vi "FuncVI2-_Call.vi"(4 "Caller CSE RefNum":T1, 5 "InstanceRef":T3, 9 "arg list":T2[](array[typedef]) {"num" format="%.2f"}) -> (0 "error out":bool, 3 "result":T2 {"num" format="%.2f"})   [LabVIEW 2021]
doc: "::: CalcExpress Toolkit :::\nCopyright (c) 2000-2026 Konstantin Shifershteyn. All rights reserved."
uses:
  cetypes.llb/CalcExpress Function Argument Info.ctl
  cetypes.llb/CalcExpress Instance RefNum.ctl
  cse.llb/CSE Instance RefNum.ctl
panel:
  in  "max arg num":i32=1000
  in  "min arg num":i32=1
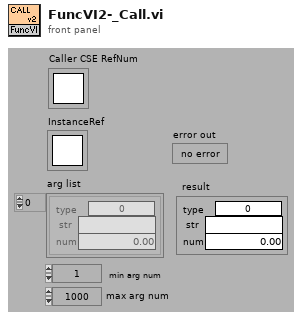
[diagram p1: front panel]
types:
  T1 = typedef "CSE Instance RefNum.ctl" = refnum<k1>
  T2 = typedef "CalcExpress Function Argument Info.ctl" = cluster{"type":u32, "str":string, "num":dbl}
  T3 = typedef "CalcExpress Instance RefNum.ctl" = refnum<k1>
  T4 = enum32{"String", "DBL Number", "identifier", "1D Array of DBL", "2D Array of DBL", "CDB Number", "1D Array of CDB", "2D Array of CDB", "1D Array of String", "2D Array of String", "Unknown data type"}
  T5 = typedef "VarMan Variable Context Handle.ctl" = i32
  T6 = typedef "CSE Callback VI RefNum.ctl" = refnum<vi>
  T7 = cluster{"type: use this constant to specify a predefined type code":enum32{"String", "DBL Number", "identifier", "1D Array of DBL", "2D Array of DBL", "CDB Number", "1D Array of CDB", "2D Array of CDB", "1D Array of String", "2D Array of String", "Unknown data type"}, string, "return value":dbl}
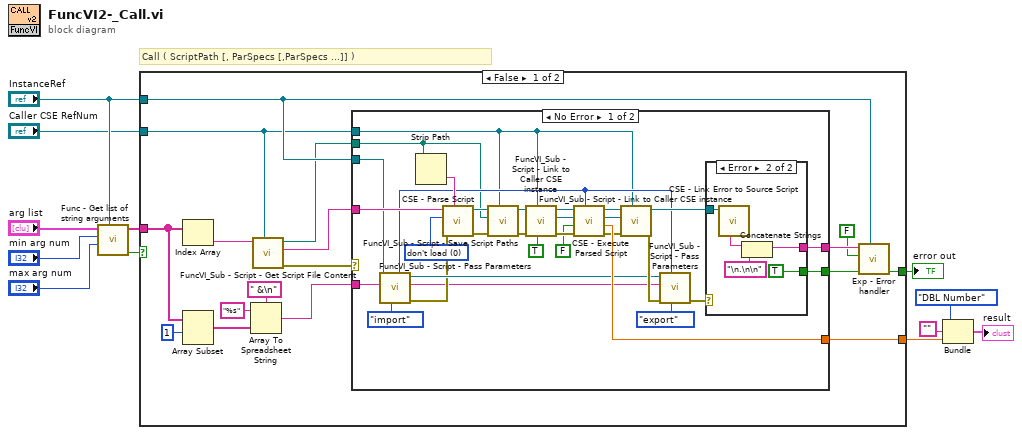
[diagram p0: block diagram]
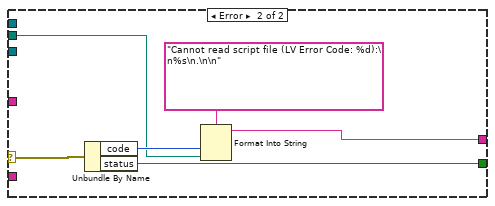
[diagram p3: hidden frame]
diagram:
  # "Call ( ScriptPath [, ParSpecs [,ParSpecs ...]] )"
  n1 = call "Func - Get list of string arguments.vi"("InstanceRef"="InstanceRef", "max arg num"="max arg num", "min arg num"="min arg num", "arg list"="arg list") -> ("error out"=w7:bool, "val list"=w8:string[])  [unwired: 4 in]
  n2 = case shown="False" w7 {
    selector: w7 -> [_ w72]
    tunnel: "InstanceRef" -> [w24 _]
    tunnel: w8 -> [w23 _]
    tunnel: [w28 w72] -> w6
    tunnel: [w29 _] -> w2
    tunnel: "Caller CSE RefNum" -> [w13 _]
    frame False {
      n3 = Index Array(array=w23) -> (element=w14:string)  [unwired: 1 in]
      n4 = Array Subset(array=w23, index=1) -> (w19:string[])  [unwired: 1 in]
      n5 = Array To Spreadsheet String(delimiter (Tab)=" &\n", array=w19, 3:"%s" ("format string")) -> (spreadsheet string=w18:string)
      n6 = call "FuncVI_Sub - Script - Get Script File Content.vi"("Caller CSE RefNum"=w13, "Script name"=w14) -> ("error out"=w17:errorcluster, "Script body"=w16:string, "Script Path"=w15:path)  [unwired: 7 in]
      n7 = case shown="No Error" w17 {
        selector: w17 -> [_ w71]
        tunnel: w16 -> [w60 _]
        tunnel: [w59 _] -> w29
        tunnel: [w57 w69] -> w27
        tunnel: w15 -> [w31 w66]
        tunnel: [w58 w68] -> w26
        tunnel: w13 -> [w32 _]
        tunnel: w18 -> [w39 _]
        tunnel: w24 -> [w38 _]
        frame No Error {
          w56 = u32 0 items=["don't load", "load", "load & test"] ("load FuncVIs")
          n8 = call "FuncVI_Sub - Script - Pass Parameters.vi"("action"=enum32{"import", "export"}."import", "parateters specifier"=w39, "CE InstanceRef"=w38) -> ("error out"=w42:errorcluster, "dup parateters specifier"=w40:string, "dup CE InstanceRef"=w43:T3, "Local VC Handle out"=w41:T5)  [unwired: 5 in]
          n9 = Strip Path(path=w31) -> (name=w55:string)  [unwired: 1 out]
          n10 = call "CSE - Parse Script.vi"("Script name"=w55, "error in"=w42, "load FuncVIs"=w56, "Script"=w60) -> ("error out"=w36:errorcluster, "CSE RefNum"=w33:T1)  [unwired: 3 in, 3 out]
          n11 = call "FuncVI_Sub - Script - Save Script Paths.vi"("Caller CSE RefNum"=w32, "error in"=w36, "Script File Path"=w31, "CSE RefNum"=w33) -> ("error out"=w35:errorcluster, "dup CSE RefNum"=w34:T1)  [unwired: 6 in]
          n12 = call "FuncVI_Sub - Script - Link to Caller CSE instance.vi"("Link(T)/Delink(F)"=TRUE, "Caller CSE RefNum"=w32, "error in"=w35, "CSE RefNum"=w34) -> ("error out"=w49:errorcluster, "Callback VI RefNum out"=w50:T6, "dup CSE RefNum"=w51:T1)  [unwired: 5 in]
          n13 = call "CSE - Execute Parsed Script.vi"("VC Handle"=w41, "error in"=w49, "Close FuncVI Refs (T)"=FALSE, "Callback VI RefNum"=w50, "CSE RefNum"=w51) -> ("error out"=w47:errorcluster, "return value"=w59:dbl, "dup Callback VI RefNum"=w52:T6, "dup CSE RefNum"=w54:T1)  [unwired: 2 in, 1 out]
          n14 = call "FuncVI_Sub - Script - Link to Caller CSE instance.vi"("Caller CSE RefNum"=w32, "error in"=w47, "Callback VI RefNum"=w52, "CSE RefNum"=w54) -> ("error out"=w45:errorcluster, "dup CSE RefNum"=w53:T1)  [unwired: 5 in, 1 out]
          n15 = call "FuncVI_Sub - Script - Pass Parameters.vi"("action"=enum32{"import", "export"}."export", "Local VC Handle"=w41, "error in"=w45, "parateters specifier"=w40, "CE InstanceRef"=w43) -> ("error out"=w46:errorcluster)  [unwired: 3 in, 3 out]
          n16 = case shown="Error" w46 {
            tunnel: w53 -> [_ w65]
            tunnel: [_ TRUE] -> w57
            tunnel: [_ w61] -> w58
            frame No Error {
            }
            frame Error {
              n17 = call "CSE - Link Error to Source Script.vi"("CSE RefNum"=w65) -> ("Error Message"=w63:string)  [unwired: 4 in, 6 out]
              n18 = Concatenate Strings(w63, "\n.\n\n" ("string")) -> (w61:string)
            }
          }
        }
        frame Error {
          n19 = Unbundle By Name(w71) -> ("code"=w67:i32, "status"=w69:bool)
          n20 = Format Into String(format string="Cannot read script file (LV Error Code: %d):\n%s\n.\n\n", w67, w66) -> (resulting string=w68:string)  [unwired: 2 in, 1 out]
        }
      }
      n21 = call "Exp - Error handler.vi"("InstanceRef"=w24, "error in"=w27, "add FuncName (T)"=FALSE, "error message in"=w26) -> ("error out"=w28:bool)  [unwired: 5 in, 2 out]
    }
    frame True {
    }
  }
  "error out" <- w6
  n22 = Bundle("type: use this constant to specify a predefined type code"=T4."DBL Number", "", "return value"=w2) -> (→"result":T7)  [unwired: 1 in]
